vi "getDetectionsB.vi"(0 "dl in":refnum<class "dl.lvclass">, 1 "bbCounts":i32[](array[numeric]), 5 "error in (no error)":errorcluster) -> (14 "dl out":refnum<class "dl.lvclass">, 15 "succBB":i32, 16 "detectionsBuffer":T2[](array[typedef]), 17 "totalDetectedBB":i32, 18 "BatchDetections":T1[](array[typedef]), 19 "error out":errorcluster)   [LabVIEW 2025, in "dl.lvlib" / "dl.lvclass"]
doc: "Parse Detection Results (Bounding Boxes)\n\nInput:\n- `bbCounts`: Number of detected bounding boxes per image, returned by `runDetectionB`.\n\nOutputs:\n- `succBB`: Parsing status. `0` indicates success; any other value indicates an error.\n- `detectionsBuffer`: Flattened 1D array containing all detected bounding boxes across the batch.\n- `totalDetectedBB`: Total number of detected bounding boxes across the batch.\n- `BatchDetections`: Detection results organized by image, with each image containing its own array of bounding boxes."
uses:
  dl.lvclass
  detect.ctl
  def/ImageDetections.ctl
  dl.lvclass/dl.ctl
  acc9ae91-1551-4c57-880a-2ffe316e0752.vi
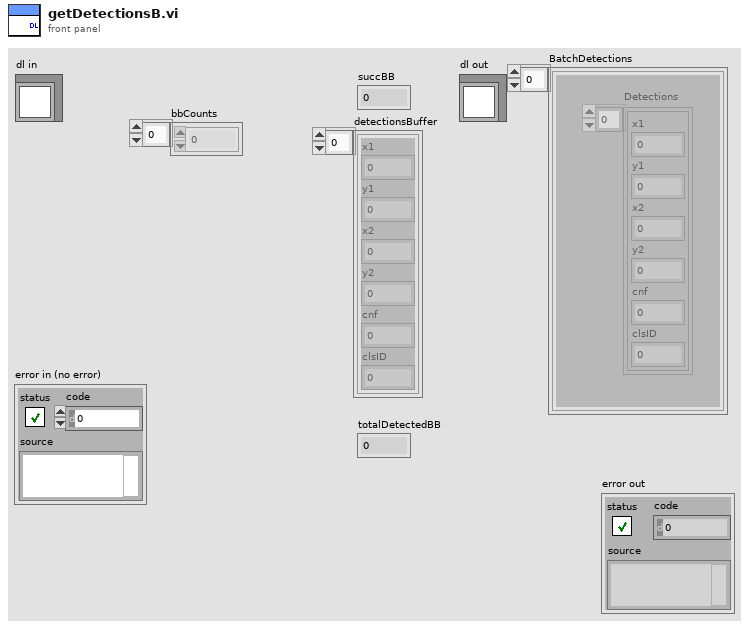
[diagram p1: front panel]
types:
  T1 = typedef "dl.lvlib/dl.lvclass/ImageDetections.ctl" = cluster{"Detections":T2[]}
  T2 = typedef "dl.lvlib/dl.lvclass/detect.ctl" = cluster{"x1":sgl, "y1":sgl, "x2":sgl, "y2":sgl, "cnf":sgl, "clsID":i32}
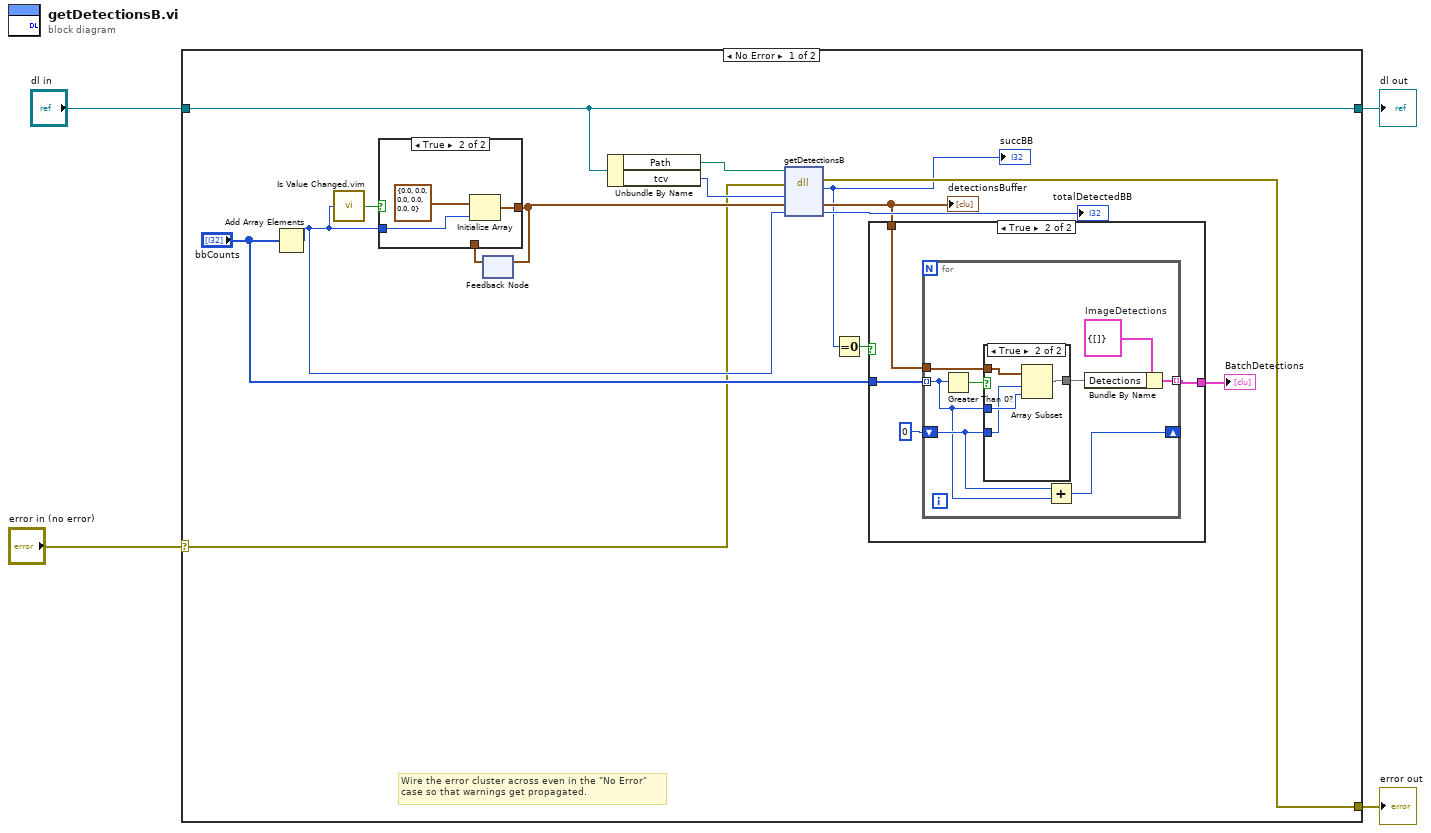
[diagram p0: block diagram]
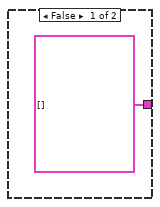
[diagram p2: hidden frame]
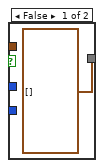
[diagram p3: hidden frame]
diagram:
  n1 = case shown="No Error" "error in (no error)" {
    selector: "error in (no error)" -> [w6 w43]
    tunnel: [w11 w43] -> w4
    tunnel: [w17 w42] -> w2
    tunnel: "dl in" -> [w17 w42]
    frame No Error {
      # "Wire the error cluster across even in the \"No Error\"\ncase so that warnings get propagated."
      n2 = Add Array Elements(numeric array="bbCounts") -> (sum=w13:i32)
      n3 = call "Is Value Changed.vim"("value"=w13) -> ("changed or first call?"=w18:bool)
      n4 = feedback #1() -> (w19:T2[])  [unwired: 1 in]
      n5 = case shown="True" w18 {
        tunnel: w13 -> [_ w40]
        tunnel: [w38 w39] -> w14
        tunnel: w19 -> [w38 _]
        frame False {
        }
        frame True {
          n6 = Initialize Array(T2 {"x1"=0.0, "y1"=0.0, "x2"=0.0, "y2"=0.0, "cnf"=0.0, "clsID"=0} ("detect"), w40) -> (w39:T2[])
        }
      }
      n7 = feedback-in #1(w14) -> ()
      n8 = Unbundle By Name(w17) -> ("Path"=w16:path, "tcv"=w15:u64)
      n9 = dll-call lib="D:/Test/adslvPackageDev/Resources/TCV_Lib.dll" fn="getDetectionsB"(path in=w16, error in=w6, "tcv"=w15, "detectionsBuffer"=w14, "totalDtectedbb"=w13) -> (error out=w11:errorcluster, "succBB"=w7:i32, "detectionsBuffer"=w9:T2[], "totalDtectedbb"=→"totalDetectedBB":i32)  [unwired: 2 in, 1 out]
      "succBB" <- w7
      "detectionsBuffer" <- w9
      n10 = Equal To 0?(x=w7) -> (x = 0?=w8:bool)
      n11 = case shown="True" w8 {
        tunnel: "bbCounts" -> [_ w24]
        tunnel: w9 -> [_ w22]
        tunnel: [T1[] [] w21] -> w5
        frame False {
        }
        frame True {
          n12 = for {
            tunnel: w24 -> [w29] mode=indexing
            shift-right: [w28] -> _
            shift-left: 0 ("bbOffset") -> [w30]
            tunnel: w22 -> [w31]
            tunnel: [w26] -> w21 mode=indexing
            w25 = T1 {"Detections"=[]}  # ImageDetections
            n13 = Greater Than 0?(x=w29) -> (x > 0?=w32:bool)
            n14 = case shown="True" w32 {
              tunnel: w31 -> [_ w37]
              tunnel: w30 -> [_ w34]
              tunnel: w29 -> [_ w36]
              tunnel: [T2[] [] w35] -> w27
              frame False {
              }
              frame True {
                n15 = Array Subset(array=w37, index=w34, length=w36) -> (w35:T2[])
              }
            }
            n16 = Add(x=w30, y=w29) -> (x+y=w28:i32)
            n17 = Bundle By Name(cluster=w25, "Detections"=w27) -> (w26:T1)
          }
        }
      }
      "BatchDetections" <- w5
    }
    frame Error {
    }
  }
  "error out" <- w4
  "dl out" <- w2
